vi "Error Handler.vi"(8 "Return Code":u32(ring)=12288 items=["FGSTATUS_UNKNOWN_ERROR"=16383, "FGSTATUS_HANDLE_DOES_NOT_MATCH_CONFIG"=12310, "FGSTATUS_CALLBACK_NOT_ASSIGNED"=12309, "FGSTATUS_VALUE_HAS_NO_SELECTOR"=12308, "FGSTATUS_WRONG_PARAMETERS_SECTION"=12307, "FGSTATUS_NO_REQUIRED_PARAMETERS_SECTION"=12306, "FGSTATUS_INVALID_VALUES_FILE"=12305, "FGSTATUS_XML_FILE_NOT_LOADED"=12304, "FGSTATUS_COULD_NOT_STOP"=12303, "FGSTATUS_COULD_NOT_START"=12302, "FGSTATUS_OUT_OF_RANGE_ADDRESS"=12301, "FGSTATUS_GENICAM_EXCEPTION"=12300, "FGSTATUS_WRONG_PARAMETER_TYPE"=12299, "FGSTATUS_WRONG_PARAMETER_NAME"=12298, "FGSTATUS_MEMORY_ERROR"=12297, "FGSTATUS_MAX_CONNECTIONS"=12296, "FGSTATUS_INVALID_VALUE"=12295, "FGSTATUS_CONFIG_NOT_LOADED"=12294, "FGSTATUS_FILE_READ_ERROR"=12293, "FGSTATUS_FILE_NOT_FOUND"=12292, "FGSTATUS_BUSY"=12291, "FGSTATUS_HW_NOT_FOUND"=12290, "FGSTATUS_UNKNOWN_HANDLE"=12289, "FGSTATUS_OK"=12288], 11 "Error In":errorcluster) -> (3 "Error Out":errorcluster)   [LabVIEW 2023, in "KYFGLib_lv.lvlib"]
uses:
  KYFGLib_lv.lvlib
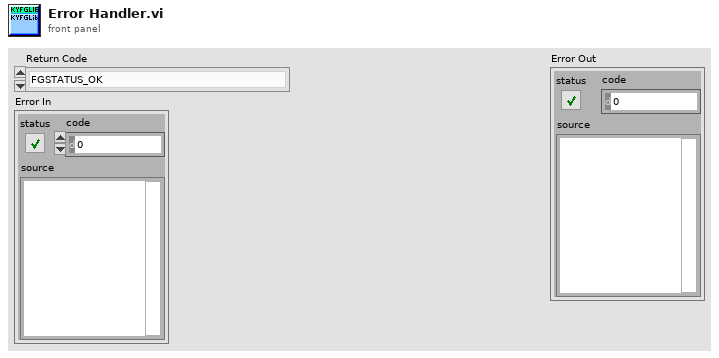
[diagram p1: front panel]
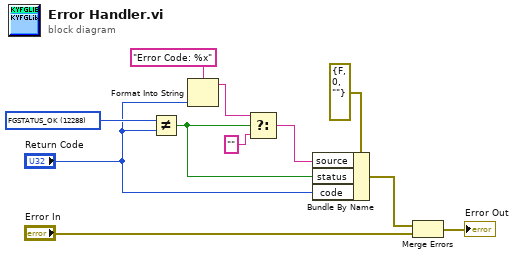
[diagram p0: block diagram]
diagram:
  w8 = u32 12288 items=["FGSTATUS_UNKNOWN_ERROR"=16383, "FGSTATUS_FEATURE_NOT_IMPLEMENTED"=16382, "FGSTATUS_FACILITY_DISABLED"=16381, "FGSTATUS_UPDATE_WRONG_BOARD_ID"=13057, "FGSTATUS_UPDATE_WRONG_VID"=13056, "FGSTATUS_CAMERA_NODES_NOT_INITIALIZED"=12800, "FGSTATUS_CAMERA_NOT_OPENED"=12553, "FGSTATUS_GRABBER_NOT_OPENED"=12552, "FGSTATUS_CAMERA_NOT_CONNECTED"=12551, "FGSTATUS_BUFFER_ALREADY_IN_INPUT_QUEUE"=12550, "FGSTATUS_STREAM_NOT_CREATED"=12549, "FGSTATUS_INVALID_STREAM_BUFFER_INFO_CMD"=12548, "FGSTATUS_INVALID_STREAM_INFO_CMD"=12547, "FGSTATUS_DESTINATION_QUEUE_NOT_SUPPORTED"=12546, "FGSTATUS_QUEUED_BUFFERS_NOT_SUPPORTED"=12545, "FGSTATUS_EXCEEDED_MAX_CAMERA_CONNECTIONS"=12544, "FGSTATUS_OPERATION_BLOCKED"=12325, "FGSTATUS_OPERATION_TIMEOUT"=12324, "FGSTATUS_UNSUPPORTED_PARAMETER_TYPE"=12323, "FGSTATUS_BUFFER_MEMORY_OVERLAP"=12322, "FGSTATUS_COULD_NOT_STOP_STREAM"=12321, "FGSTATUS_FILE_CREATE_ERROR"=12320, "FGSTATUS_NO_PARAMETER_TYPE"=12319, "FGSTATUS_ROOT_IS_NOT_OBJECT"=12318, "FGSTATUS_CAMERA_OR_GRABBER_SECTION_NOT_ARRAY"=12317, "FGSTATUS_WRONG_SCHEMA_VERSION"=12316, "FGSTATUS_CANNOT_START_HW_STREAM"=12315, "FGSTATUS_PARAMETER_NOT_WRITABLE"=12314, "FGSTATUS_GRABBER_FIRMWARE_NOT_SUPPORTED"=12313, "FGSTATUS_BUFFER_UNSUPPORTED_SIZE"=12312, "FGSTATUS_BUFFER_TOO_SMALL"=12311, "FGSTATUS_HANDLE_DOES_NOT_MATCH_CONFIG"=12310, "FGSTATUS_CALLBACK_NOT_ASSIGNED"=12309, "FGSTATUS_VALUE_HAS_NO_SELECTOR"=12308, "FGSTATUS_WRONG_PARAMETERS_SECTION"=12307, "FGSTATUS_NO_REQUIRED_PARAMETERS_SECTION"=12306, "FGSTATUS_INVALID_VALUES_FILE"=12305, "FGSTATUS_XML_FILE_NOT_LOADED"=12304, "FGSTATUS_COULD_NOT_STOP"=12303, "FGSTATUS_COULD_NOT_START"=12302, "FGSTATUS_OUT_OF_RANGE_ADDRESS"=12301, "FGSTATUS_GENICAM_EXCEPTION"=12300, "FGSTATUS_WRONG_PARAMETER_TYPE"=12299, "FGSTATUS_WRONG_PARAMETER_NAME"=12298, "FGSTATUS_MEMORY_ERROR"=12297, "FGSTATUS_MAX_CONNECTIONS"=12296, "FGSTATUS_INVALID_VALUE"=12295, "FGSTATUS_CONFIG_NOT_LOADED"=12294, "FGSTATUS_FILE_READ_ERROR"=12293, "FGSTATUS_FILE_NOT_FOUND"=12292, "FGSTATUS_BUSY"=12291, "FGSTATUS_HW_NOT_FOUND"=12290, "FGSTATUS_UNKNOWN_HANDLE"=12289, "FGSTATUS_OK"=12288] ("Ring")
  n1 = Not Equal?(x=w8, y="Return Code") -> (x != y?=w5:bool)
  n2 = Format Into String(format string="Error Code: %x", "Return Code") -> (resulting string=w10:string)  [unwired: 2 in, 1 out]
  n3 = Select(t=w10, s=w5, f="" ("format string")) -> (s? t:f=w6:string)
  n4 = Bundle By Name(cluster=errorcluster {"status"=FALSE, "code"=0, "source"=""} ("error constant"), "source"=w6, "status"=w5, "code"="Return Code") -> (w2:errorcluster)
  n5 = Merge Errors(w2, "Error In") -> (→"Error Out":errorcluster)
